vi "Range-check.vi"(6 "超时时间（Ms）":dbl, 7 "枚举":enum16{"Reset", "usage"}(ring)=enum."usage", 8 "设定值下限":dbl, 9 "设定值上限":dbl, 10 "变量":dbl, 11 "设定时间MS":dbl) -> (2 "成功？":bool, 3 "Time has Elapsed":bool caption="超时？")   [LabVIEW 2018]
panel:
  out "Elapsed Time (s)":dbl caption="已用时间(s)"
  # "功能说明：\n在一定的时间范围内，监测目标值在设置的时间内维持住规定的时间\n1.需外接循环使用\n2.需先执行一次初始化\n3.由于使用移位寄存器导致不能重入\n4.如需重入执行可选择：\n    a.复制本VI并重命名，分开调用\n    b.修改内部初始化机制，每次Usage分支都输入设定值"
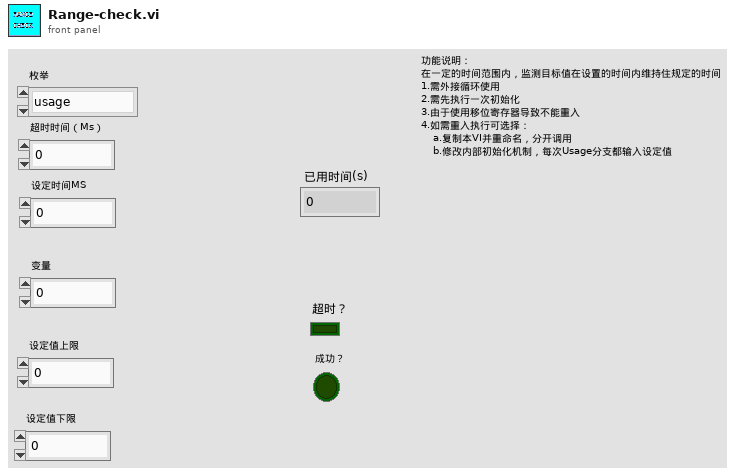
[diagram p1: front panel]
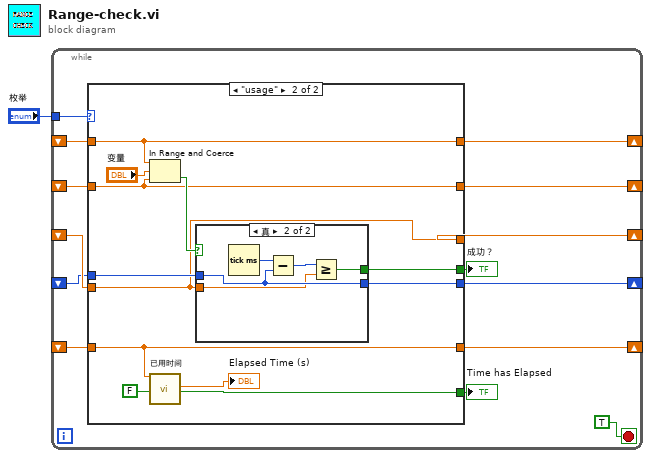
[diagram p0: block diagram]
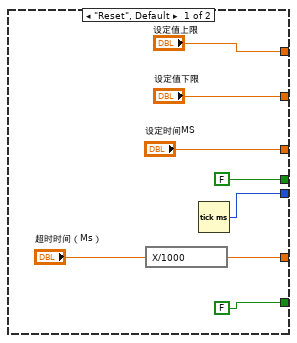
[diagram p2: hidden frame]
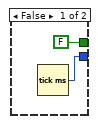
[diagram p3: hidden frame]
diagram:
  n1 = while {
    shift-right: [w11] -> _
    shift-left: _ -> [w10]
    tunnel: "枚举" -> [w12]
    shift-right: [w7] -> _
    shift-left: _ -> [w13]
    shift-right: [w6] -> _
    shift-left: _ -> [w15]
    shift-right: [w5] -> _
    shift-left: _ -> [w14]
    shift-right: [w2] -> _
    shift-left: _ -> [w9]
    stop <- TRUE stop-if-true
    n2 = case shown="\"usage\"" w12 {
      tunnel: w15 -> [_ w26]
      tunnel: w14 -> [_ w27]
      tunnel: w13 -> [_ w28]
      tunnel: [w23 w30] -> w11
      tunnel: w10 -> [_ w31]
      tunnel: w9 -> [_ w24]
      tunnel: [FALSE w29] -> w8
      tunnel: ["设定时间MS" w28] -> w7
      tunnel: ["设定值上限" w26] -> w6
      tunnel: ["设定值下限" w27] -> w5
      tunnel: [FALSE ("Time has Elapsed") w25] -> w3
      tunnel: [w16 w24] -> w2
      frame "Reset", Default {
        n3 = expression code="X/1000"("超时时间（Ms）") -> (w16:dbl)
        n4 = Tick Count (ms)() -> (millisecond timer value=w23:u32)
      }
      frame "usage" {
        n5 = In Range and Coerce(upper limit=w26, x="变量", lower limit=w27) -> (In Range?=w34:bool)  [unwired: 1 out]
        n6 = call "已用时间"("Time Target (s)"=w24, "Auto Reset"=FALSE) -> ("Elapsed Time (s)"=→"Elapsed Time (s)":dbl, "Time has Elapsed"=w25:bool)  [unwired: 10 in, 6 out]
        n7 = case shown="真" w34 {
          tunnel: w31 -> [_ w41]
          tunnel: [w37 w41] -> w30
          tunnel: w28 -> [_ w39]
          tunnel: [FALSE w38] -> w29
          frame False {
            n8 = Tick Count (ms)() -> (millisecond timer value=w37:u32)
          }
          frame True {
            n9 = Tick Count (ms)() -> (millisecond timer value=w42:u32)
            n10 = Subtract(x=w42, y=w41) -> (x-y=w40:u32)
            n11 = Greater Or Equal?(x=w40, y=w39) -> (x >= y?=w38:bool)
          }
        }
      }
    }
    "成功？" <- w8
    "Time has Elapsed" <- w3
  }
